vi "DrivePlanPath.vi"(1 "DrivePathPlanParams":T1={"max_velocity (in/s)"=100.0, "max_acceleration (in/s^2)"=80.0, "max_jerk (in/s^3)"=100.0, "dt(ms)"=40, "sample_count"=1000, "wheelbase_width (in)"=25.0} {"dt(ms)" items=["TrajectoryDuration_0ms"=0, "TrajectoryDuration_5ms"=5, "TrajectoryDuration_10ms"=10, "TrajectoryDuration_20ms"=20, "TrajectoryDuration_30ms"=30, "TrajectoryDuration_40ms"=40, "TrajectoryDuration_50ms"=50, "TrajectoryDuration_100ms"=100]}, 2 "DrivePlanRequest":T3) -> (0 "DrivePlanResponse":T6)   [LabVIEW 2017]
uses:
  PathPlannerSupport/TypeDefs/DrivePlanResponse.ctl
  Pathfinder/Pathfinder-LabVIEW/Pathfinder-Lib/VIs/Segment.ctl
  PathPlannerSupport/TypeDefs/DrivePlanRequest.ctl
  TypeDef/AutoWaypointType.ctl
  Pathfinder/Pathfinder-LabVIEW/Pathfinder-Lib/VIs/Waypoint.ctl
  PathPlannerSupport/TypeDefs/DrivePathfinderParams.ctl
  <vilib>/Rock Robotics/WPI/ThirdParty/Phoenix-LabVIEW/Motor Controller/Controls/CTRE_Phoenix_MotorControl_TrajectoryPointTimeDur.ctl
  Pathfinder/Pathfinder-LabVIEW/Pathfinder-Lib/Pathfinder.lvlib
panel:
  out "Error Scenario":string
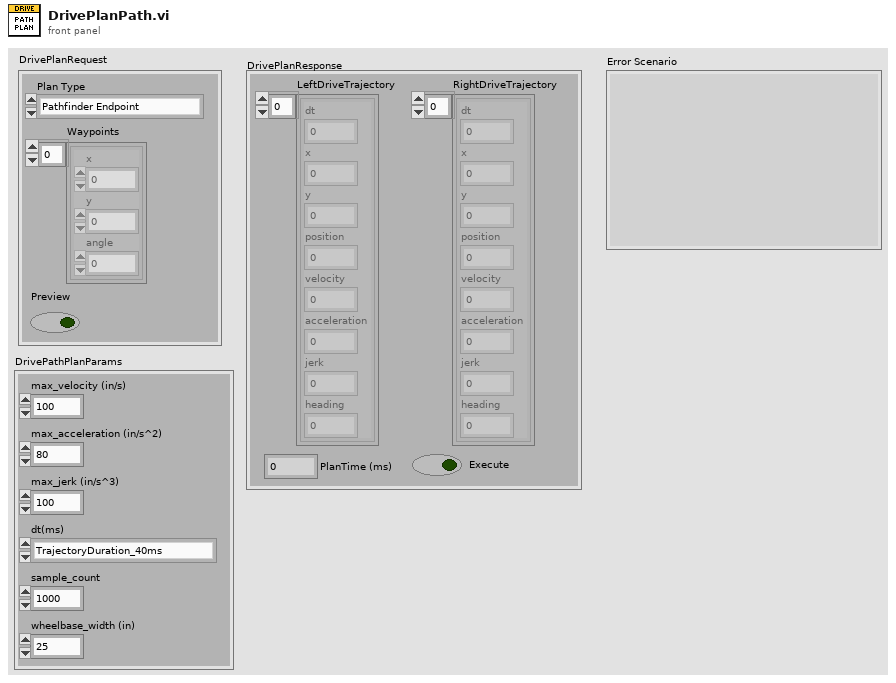
[diagram p1: front panel]
types:
  T1 = typedef "DrivePathfinderParams.ctl" = cluster{"max_velocity (in/s)":dbl, "max_acceleration (in/s^2)":dbl, "max_jerk (in/s^3)":dbl, "dt(ms)":T2, "sample_count":i32, "wheelbase_width (in)":dbl}
  T2 = typedef "CTRE_Phoenix_MotorControl_TrajectoryPointTimeDur.ctl" = i32
  T3 = typedef "DrivePlanRequest.ctl" = cluster{"Plan Type":T4, "Waypoints":T5[], "Preview":bool}
  T4 = typedef "AutoWaypointType.ctl" = enum16{"Pathfinder Endpoint", "Pathfinder Waypoint", "Zero-Radius Turn Endpoint", "Stationary", "Vision Assist Endpoint", "Stop"}
  T5 = typedef "Pathfinder.lvlib/Waypoint.ctl" = cluster{"x":dbl, "y":dbl, "angle":dbl}
  T6 = typedef "DrivePlanResponse.ctl" = cluster{"LeftDriveTrajectory":T7[], "RightDriveTrajectory":T7[], "PlanTime (ms)":u32, "Execute":bool}
  T7 = typedef "Pathfinder.lvlib/Segment.ctl" = cluster{"dt":dbl, "x":dbl, "y":dbl, "position":dbl, "velocity":dbl, "acceleration":dbl, "jerk":dbl, "heading":dbl}
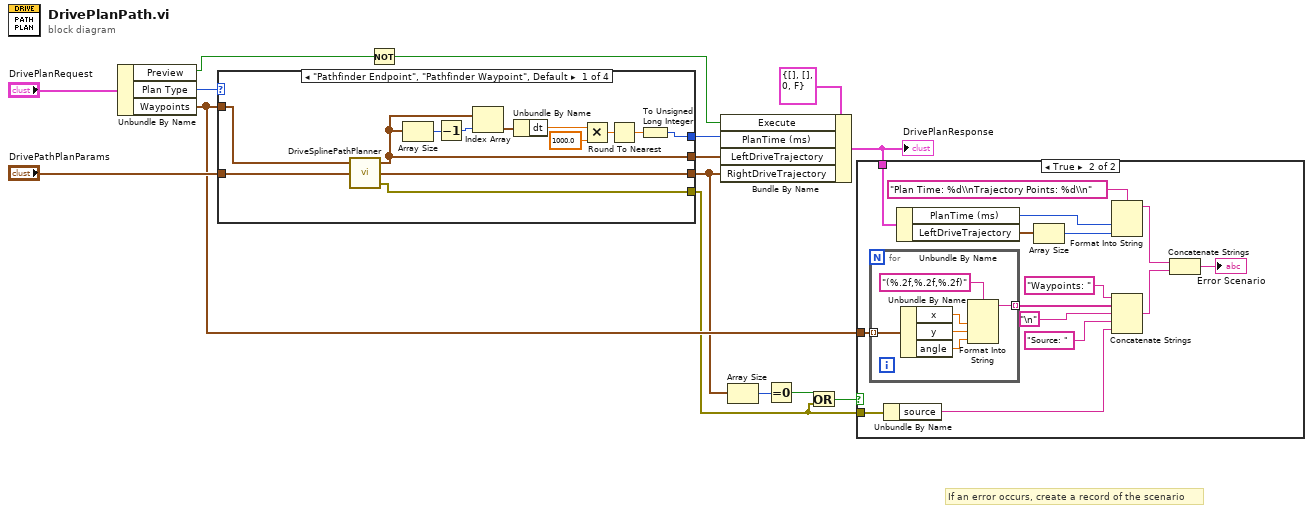
[diagram p0: block diagram]
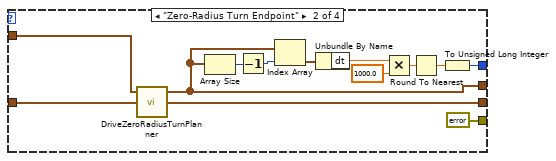
[diagram p3: hidden frame]
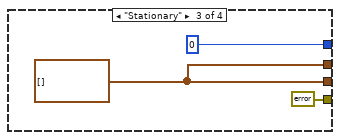
[diagram p4: hidden frame]
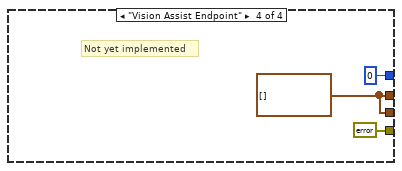
[diagram p5: hidden frame]
diagram:
  # "If an error occurs, create a record of the scenario"
  n1 = Unbundle By Name("DrivePlanRequest") -> ("Preview"=w11:bool, "Plan Type"=w15:T4, "Waypoints"=w6:T5[])
  n2 = case shown="\"Pathfinder Endpoint\", \"Pathfinder Waypoint\", Default" w15 {
    tunnel: "DrivePathPlanParams" -> [w28 w41 _ _]
    tunnel: [w25 w30 w44 w46] -> w9
    tunnel: [w27 w39 w44 w46] -> w5
    tunnel: [w18 w31 u32 0 ("PlanTime (ms)") u32 0 ("PlanTime (ms)")] -> w8
    tunnel: w6 -> [w17 w40 _ _]
    tunnel: [w16 errorcluster {"status"=FALSE, "code"=0, "source"=""} ("error out") errorcluster {"status"=FALSE, "code"=0, "source"=""} ("error out") errorcluster {"status"=FALSE, "code"=0, "source"=""} ("error out")] -> w1
    frame "Pathfinder Endpoint", "Pathfinder Waypoint", Default {
      n3 = call "DriveSplinePathPlanner.vi"("DrivePathPlanParams"=w28, "path"=w17) -> ("error out"=w16:errorcluster, "RightTrajectory"=w27:T7[], "LeftTrajectory"=w25:T7[])  [unwired: 1 in]
      n4 = Array Size(array=w25) -> (size(s)=w26:i32)
      n5 = Decrement(x=w26) -> (x-1=w24:i32)
      n6 = Index Array(array=w25, index=w24) -> (element=w23:T7)
      n7 = Unbundle By Name(w23) -> ("dt"=w22:dbl)
      n8 = Multiply(x=w22, y=1000.0) -> (x*y=w20:dbl)
      n9 = Round To Nearest(number=w20) -> (nearest integer value=w19:dbl)
      n10 = To Unsigned Long Integer(number=w19) -> (unsigned 32bit integer=w18:u32)
    }
    frame "Zero-Radius Turn Endpoint" {
      n11 = call "DriveZeroRadiusTurnPlanner.vi"("DrivePathPlanParams"=w41, "Waypoints"=w40) -> ("RightTrajectory"=w39:T7[], "LeftTrajectory"=w30:T7[])  [unwired: 2 in]
      n12 = Array Size(array=w30) -> (size(s)=w38:i32)
      n13 = Decrement(x=w38) -> (x-1=w37:i32)
      n14 = Index Array(array=w30, index=w37) -> (element=w36:T7)
      n15 = Unbundle By Name(w36) -> ("dt"=w35:dbl)
      n16 = Multiply(x=w35, y=1000.0) -> (x*y=w33:dbl)
      n17 = Round To Nearest(number=w33) -> (nearest integer value=w32:dbl)
      n18 = To Unsigned Long Integer(number=w32) -> (unsigned 32bit integer=w31:u32)
    }
    frame "Stationary" {
      w44 = T7[] [] ("LeftTrajectory")
    }
    frame "Vision Assist Endpoint" {
      w46 = T7[] [] ("LeftTrajectory")
      # "Not yet implemented"
    }
  }
  n19 = Not(x=w11) -> (.not. x?=w10:bool)
  n20 = Bundle By Name(cluster=T6 {"LeftDriveTrajectory"=[], "RightDriveTrajectory"=[], "PlanTime (ms)"=0, "Execute"=FALSE} ("DrivePlanResponse"), "Execute"=w10, "PlanTime (ms)"=w8, "LeftDriveTrajectory"=w9, "RightDriveTrajectory"=w5) -> (w7:T6)
  "DrivePlanResponse" <- w7
  n21 = Array Size(array=w5) -> (size(s)=w4:i32)
  n22 = Equal To 0?(x=w4) -> (x = 0?=w3:bool)
  n23 = Or(x=w3, y=w1) -> (x .or. y?=w2:bool)
  n24 = case shown="True" w2 {
    tunnel: w7 -> [_ w62]
    tunnel: w6 -> [_ w60]
    tunnel: w1 -> [_ w48]
    frame False {
    }
    frame True {
      n25 = for {
        tunnel: w60 -> [w68] mode=indexing
        tunnel: [w63] -> w59 mode=indexing
        n26 = Unbundle By Name(w68) -> ("x"=w66:dbl, "y"=w67:dbl, "angle"=w65:dbl)
        n27 = Format Into String(format string="(%.2f,%.2f,%.2f)", w66, w67, w65) -> (resulting string=w63:string)  [unwired: 2 in, 1 out]
      }
      n28 = Unbundle By Name(w48) -> ("source"=w50:string)
      n29 = Unbundle By Name(w62) -> ("PlanTime (ms)"=w56:u32, "LeftDriveTrajectory"=w61:T7[])
      n30 = Array Size(array=w61) -> (size(s)=w55:i32)
      n31 = Format Into String(format string="Plan Time: %d\\nTrajectory Points: %d\\n", w56, w55) -> (resulting string=w54:string)  [unwired: 2 in, 1 out]
      n32 = Concatenate Strings("Waypoints: ", w59, "\n", "Source: " ("string"), w50) -> (w53:string)
      n33 = Concatenate Strings(w54, w53) -> (→"Error Scenario":string)
    }
  }
